vi "Window_Setup.vi"(0 "VI":refnum<vi>, 11 "error in":errorcluster) -> (15 "error out":errorcluster)   [LabVIEW 2020, in "GH_App.lvlib"]
doc: "Sets up the window of Main: picture \"Screen\" at the top left (moved up and left by its 3 px frame, so its drawing area starts at the window corner) with a fixed drawing area of 1280 x 720, never erasing; all other controls are moved to the right outside the visible area; the panel is sized to the screen; no title bar (the X at the top right of the screen ends the game)."
uses:
  GH_App.lvlib
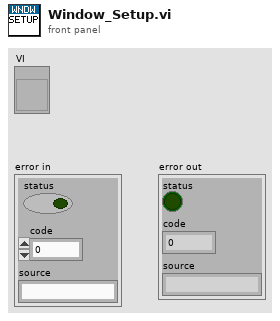
[diagram p1: front panel]
types:
  T1 = typedef "LVRectTypeDef.ctl" = cluster{"left":i16, "top":i16, "right":i16, "bottom":i16}
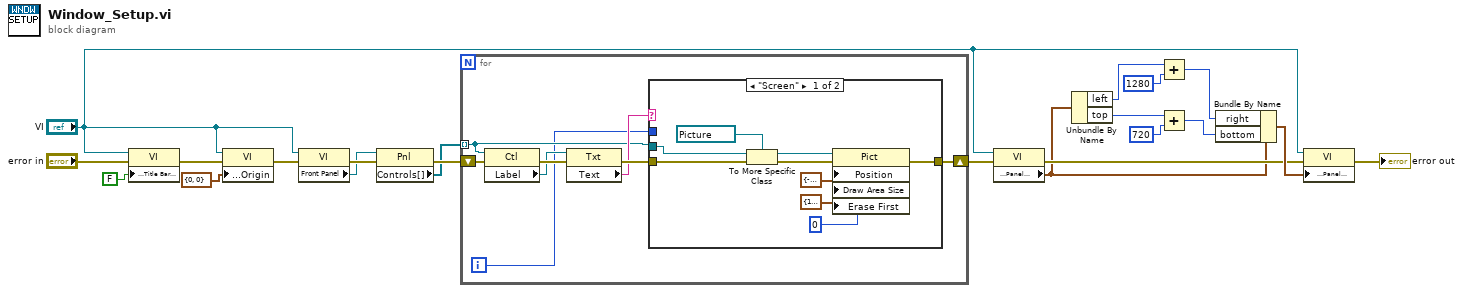
[diagram p0: block diagram]
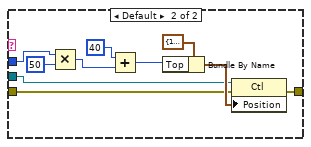
[diagram p2: hidden frame]
diagram:
  n1 = property class="VI"(reference="VI", error in="error in", "Front Panel Window:Title Bar Visible"=FALSE ("no title bar")) -> (error out=w4:errorcluster)  [unwired: 1 out]
  n2 = property class="VI"(reference="VI", error in=w4, "Front Panel Window:Origin"=cluster{"Horizontal":i16, "Vertical":i16} {"Horizontal"=0, "Vertical"=0} ("Origin")) -> (error out=w6:errorcluster)  [unwired: 1 out]
  n3 = property class="VI"(reference="VI", error in=w6) -> (error out=w8:errorcluster, "Front Panel"=w7:refnum<vi>)  [unwired: 1 out]
  n4 = property class="Pnl"(reference=w7, error in=w8) -> (error out=w10:errorcluster, "Controls[]"=w9:refnum<vi>[])  [unwired: 1 out]
  n5 = for {
    tunnel: w9 -> [w23] mode=indexing
    shift-right: [w25] -> w11
    shift-left: w10 -> [w24]
    i -> [w22]
    n6 = property class="Ctl"(reference=w23, error in=w24) -> (error out=w27:errorcluster, "Label"=w26:refnum<vi>)  [unwired: 1 out]
    n7 = property class="Txt"(reference=w26, error in=w27) -> (error out=w29:errorcluster, "Text"=w28:string)  [unwired: 1 out]
    n8 = case shown="\"Screen\"" w28 {
      tunnel: w22 -> [_ w41]
      tunnel: w23 -> [w30 w39]
      tunnel: w29 -> [w31 w40]
      tunnel: [w38 w48] -> w25
      frame "Screen" {
        n9 = To More Specific Class(target class=refnum<vi> refnum ("Picture class"), reference=w30, error in=w31) -> (specific class reference=w33:refnum<vi>, error out=w34:errorcluster)
        n10 = property class="Pict"(reference=w33, error in=w34, "Position"=cluster{"Left":i32, "Top":i32} {"Left"=-3, "Top"=-3} ("Top left minus the 3 px frame"), "Draw Area Size"=cluster{"Width":i32, "Height":i32} {"Width"=1280, "Height"=720} ("Screen size"), "Erase First"=u8 0 ("never erase")) -> (error out=w38:errorcluster)  [unwired: 1 out]
      }
      frame Default {
        n11 = Multiply(x=w41, y=50) -> (x*y=w45:i32)
        n12 = Add(x=40, y=w45) -> (x+y=w46:i32)
        n13 = Bundle By Name(cluster=cluster{"Left":i32, "Top":i32} {"Left"=1320, "Top"=40} ("right of the screen"), "Top"=w46) -> (w47:cluster{"Left":i32, "Top":i32})
        n14 = property class="Ctl"(reference=w39, error in=w40, "Position"=w47) -> (error out=w48:errorcluster)  [unwired: 1 out]
      }
    }
  }
  n15 = property class="VI"(reference="VI", error in=w11) -> (error out=w13:errorcluster, "Front Panel Window:Panel Bounds"=w12:T1)  [unwired: 1 out]
  n16 = Unbundle By Name(w12) -> ("left"=w14:i16, "top"=w15:i16)
  n17 = Add(x=w14, y=i16 1280) -> (x+y=w17:i16)
  n18 = Add(x=w15, y=i16 720) -> (x+y=w19:i16)
  n19 = Bundle By Name(cluster=w12, "right"=w17, "bottom"=w19) -> (w20:T1)
  n20 = property class="VI"(reference="VI", error in=w13, "Front Panel Window:Panel Bounds"=w20) -> (error out=→"error out":errorcluster)  [unwired: 1 out]
